vi "Refresh Feed (By URI).vi"(8 "error in (no error)":errorcluster, 11 "feed URI in":string) -> (0 "error out":errorcluster, 3 "feed URI out":string)   [LabVIEW 2014, in "NIPM_API.lvlib"]
doc: "Refreshes NI Package Manager with data from a registered feed\n\nNote: You should refresh after adding/removing packages from feeds, so that NI Package Manager will update with the latest feed and package data.\n\nINPUT(s)\n<B>Feed URI in</B>: Specifies the URI of the registered feed\n\nOUTPUT(s)\n<B>Feed URI out</B>: Outputs the specified feed URI"
uses:
  NIPM_API.lvlib
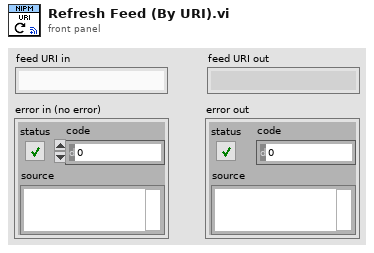
[diagram p1: front panel]
types:
  T1 = typedef "NIPM_API.lvlib/feed.ctl" = cluster{"Name":string, "URI":string}
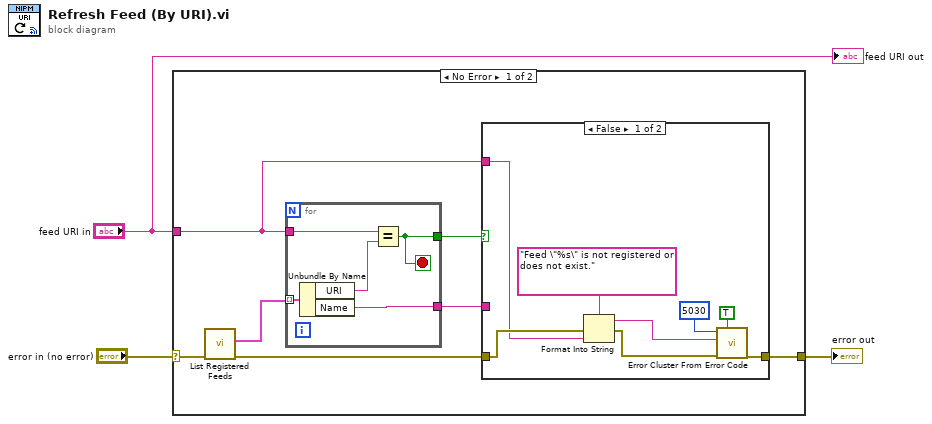
[diagram p0: block diagram]
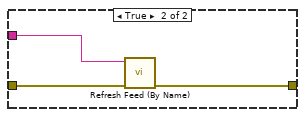
[diagram p2: hidden frame]
diagram:
  n1 = case shown="No Error" "error in (no error)" {
    selector: "error in (no error)" -> [w4 w27]
    tunnel: [w10 w27] -> w3
    tunnel: "feed URI in" -> [w7 _]
    frame No Error {
      n2 = call "List Registered Feeds.vi"("error in"=w4) -> ("error out"=w8:errorcluster, "registered feeds"=w5:T1[])  [unwired: 9 in]
      n3 = for {
        tunnel: w7 -> [w25]
        tunnel: w5 -> [w26] mode=indexing
        tunnel: [w23] -> w6
        tunnel: [w22] -> w9
        stop <- w23 stop-if-true
        n4 = Unbundle By Name(w26) -> ("URI"=w24:string, "Name"=w22:string)
        n5 = Equal?(x=w25, y=w24) -> (x = y?=w23:bool)
      }
      n6 = case shown="False" w6 {
        tunnel: w8 -> [w14 w21]
        tunnel: [w13 w20] -> w10
        tunnel: w7 -> [w12 _]
        tunnel: w9 -> [_ w19]
        frame False {
          n7 = Format Into String(format string="Feed \"%s\" is not registered or does not exist.", error in=w14, w12) -> (resulting string=w15:string, error out=w16:errorcluster)  [unwired: 1 in]
          n8 = call <vilib>:"Error Cluster From Error Code.vi"("show call chain? (False)"=TRUE, "error in (no error)"=w16, "error message (\"\")"=w15, "error code (0)"=5030) -> ("error out"=w13:errorcluster)  [unwired: 5 in]
        }
        frame True {
          n9 = call "Refresh Feed (By Name).vi"("error in"=w21, "feed name in"=w19) -> ("error out"=w20:errorcluster)  [unwired: 8 in, 1 out]
        }
      }
    }
    frame Error {
    }
  }
  "error out" <- w3
  "feed URI out" <- "feed URI in"
